vi "RemoteVI Send Client Windows.vi"(0 "Client":T1, 1 "capture?":bool, 5 "message":string, 7 "frame":string, 9 "captures":T2(array[cluster])) -> (4 "Client out":T1)   [LabVIEW 2020, in "RemoteVI.lvlib"]
doc: "The windows part (docs\\protocol.md section 7) for one client. First the list: when message (windows [...]) differs from windows sent - the list this client was last told, empty for a new client, so a client gets the list on connect - frame (message as a WebSocket text frame) is written with TCP Write (500 ms) and windows sent becomes message; a failed write sets closed. Then, when captures were made in this iteration (capture?), each window's picture goes out with RemoteVI Send Window Frame.vi against the picture of that window this client was last sent (window frames, looked up by id) - flow control and the shared seq decide, as for FRAME. window frames is rebuilt in the order of captures, so the pictures of windows that are gone are dropped; without captures it is kept. A closed client is passed through (Send Window Frame skips it too)."
uses:
  RemoteVI.lvlib
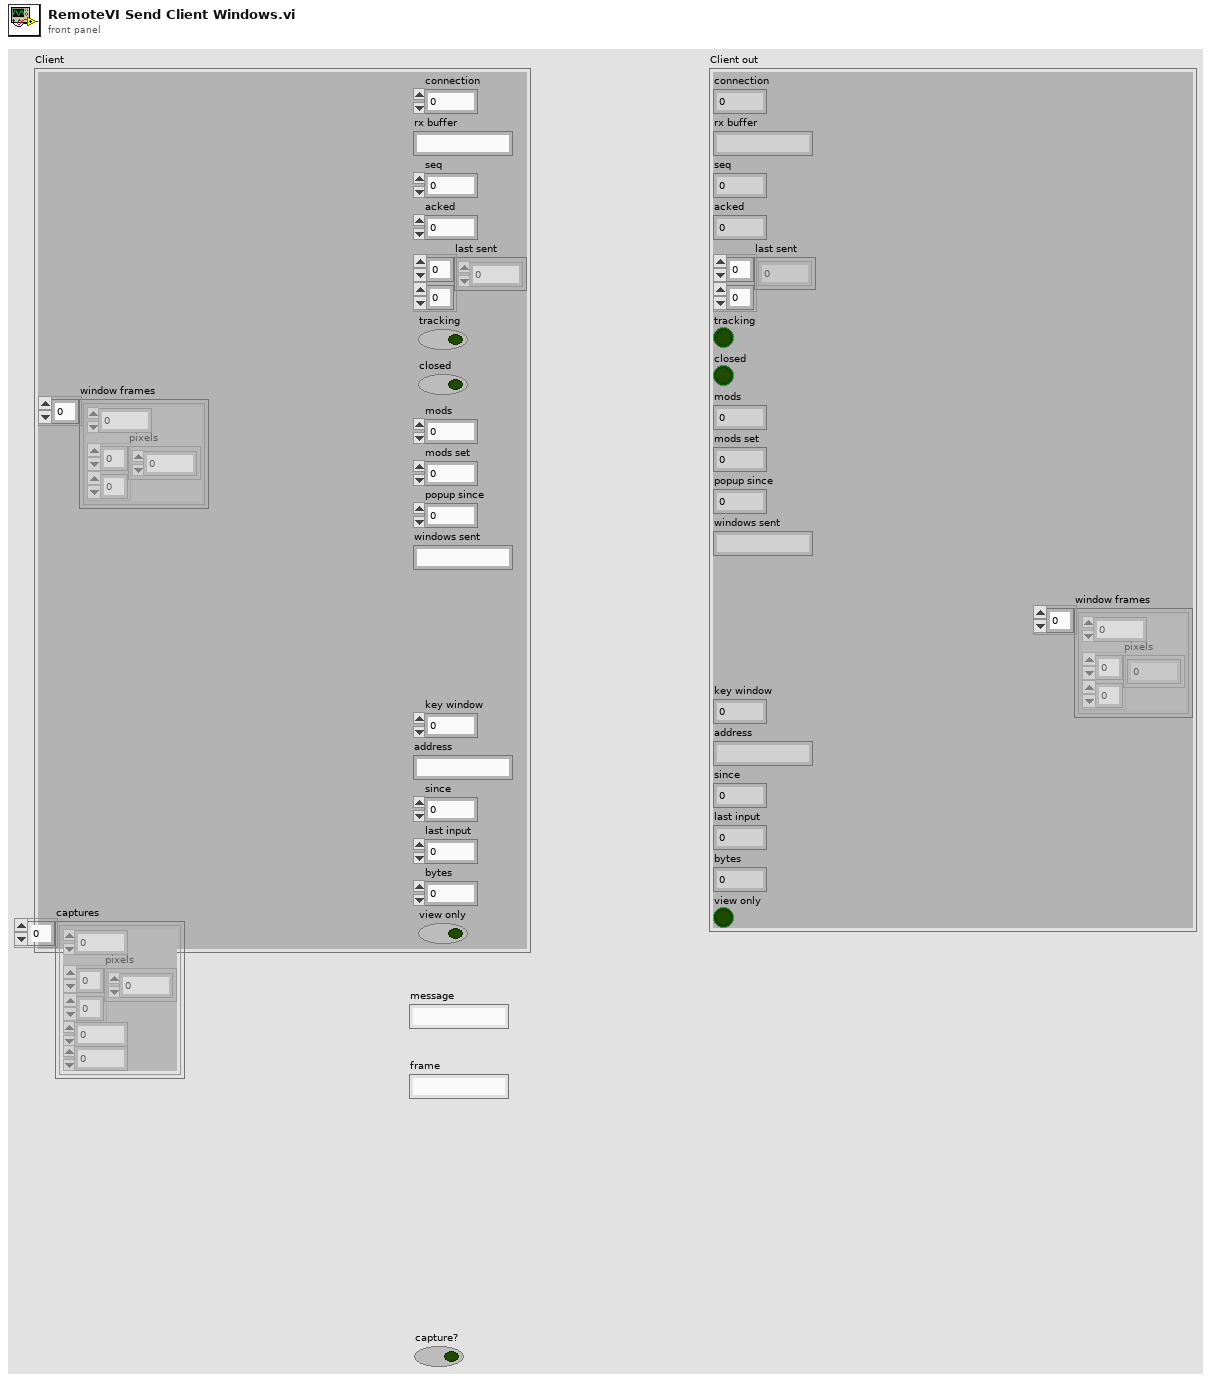
[diagram p1: front panel]
types:
  T1 = cluster{"connection":u32, "rx buffer":string, "seq":u32, "acked":u32, "last sent":u32[][], "tracking":bool, "closed":bool, "mods":u8, "mods set":u8, "popup since":u32, "windows sent":string, "window frames":cluster{"id":u64, "pixels":u32[][]}[], "key window":u64, "address":string, "since":dbl, "last input":dbl, "bytes":dbl, "view only":bool}
  T2 = cluster{"id":u64, "pixels":u32[][], "width":i32, "height":i32}[]
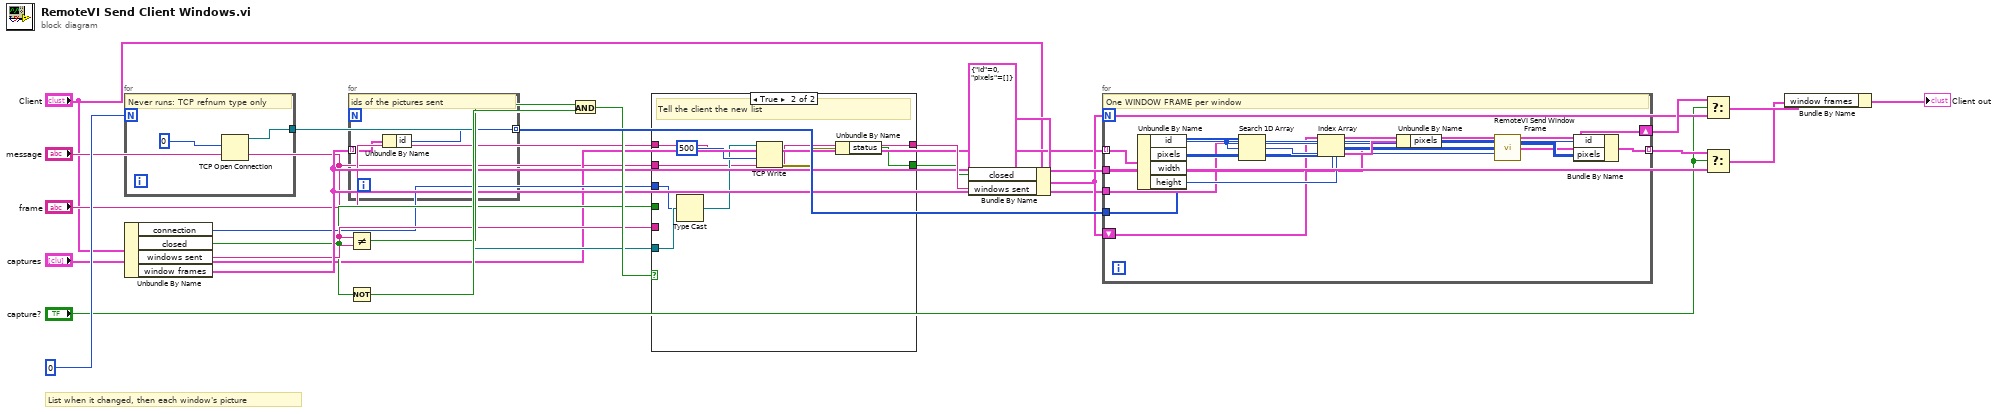
[diagram p0: block diagram]
diagram:
  # "List when it changed, then each window's picture"
  n1 = for {
    N: 0 -> [_]
    tunnel: [w26] -> w7
    # "Never runs: TCP refnum type only"
    n2 = TCP Open Connection(remote port or service name=u16 0) -> (connection ID=w26:refnum<k5>)  [unwired: 4 in, 1 out]
  }
  n3 = Unbundle By Name("Client") -> ("connection"=w8:u32, "closed"=w9:bool, "windows sent"=w10:string, "window frames"=w11:cluster{"id":u64, "pixels":u32[][]}[])
  n4 = for {
    tunnel: w11 -> [w27] mode=indexing
    tunnel: [w28] -> w18 mode=indexing
    # "ids of the pictures sent"
    n5 = Unbundle By Name(w27) -> ("id"=w28:u64)
  }
  n6 = Not Equal?(x=w10, y="message") -> (x != y?=w12:bool)
  n7 = Not(x=w9) -> (.not. x?=w13:bool)
  n8 = And(x=w12, y=w13) -> (x .and. y?=w14:bool)
  n9 = case shown="True" w14 {
    tunnel: "frame" -> [_ w32]
    tunnel: "message" -> [_ w34]
    tunnel: w8 -> [_ w31]
    tunnel: w9 -> [w29 _]
    tunnel: w10 -> [w30 _]
    tunnel: [w30 w34] -> w16
    tunnel: w7 -> [_ w33]
    tunnel: [w29 w38] -> w15
    frame False {
      # "Unchanged or closed"
    }
    frame True {
      # "Tell the client the new list"
      n10 = Type Cast(type=w33, x=w31) -> (*(type *) &x=w35:refnum<k5>)
      n11 = TCP Write(connection ID=w35, data in=w32, 9:500) -> (error out=w37:errorcluster)  [unwired: 1 in, 2 out]
      n12 = Unbundle By Name(w37) -> ("status"=w38:bool)
    }
  }
  n13 = Bundle By Name(cluster="Client", "closed"=w15, "windows sent"=w16) -> (w17:T1)
  n14 = for {
    tunnel: "captures" -> [w39] mode=indexing
    tunnel: cluster{"id":u64, "pixels":u32[][]} {"id"=0, "pixels"=[]} -> [w42]
    tunnel: w11 -> [w41]
    tunnel: w18 -> [w40]
    shift-right: [w44] -> w20
    shift-left: w17 -> [w43]
    tunnel: [w53] -> w21 mode=indexing
    # "One WINDOW FRAME per window"
    n15 = Unbundle By Name(w39) -> ("id"=w45:u64, "pixels"=w46:u32[][], "width"=w47:i32, "height"=w48:i32)
    n16 = Search 1D Array(1D array=w40, element=w45) -> (index of element=w49:i32)  [unwired: 1 in]
    n17 = Index Array(array=w41, index=w49) -> (element=w50:cluster{"id":u64, "pixels":u32[][]})
    n18 = Unbundle By Name(w50) -> ("pixels"=w51:u32[][])
    n19 = call "RemoteVI Send Window Frame.vi"("Client"=w43, "height"=w48, "last sent"=w51, "id"=w45, "pixmap"=w46, "width"=w47) -> ("Client out"=w44:T1, "last sent out"=w52:u32[][])  [unwired: 6 in, 2 out]
    n20 = Bundle By Name(cluster=w42, "id"=w45, "pixels"=w52) -> (w53:cluster{"id":u64, "pixels":u32[][]})
  }
  n21 = Select(t=w20, s="capture?", f=w17) -> (s? t:f=w23:T1)
  n22 = Select(t=w21, s="capture?", f=w11) -> (s? t:f=w22:cluster{"id":u64, "pixels":u32[][]}[])
  n23 = Bundle By Name(cluster=w23, "window frames"=w22) -> (→"Client out":T1)
